vi "poc.ip.kria.generated.vi"(10 "data valid":bool[](array[boolean])=[FALSE, FALSE, TRUE, TRUE, TRUE, FALSE, FALSE, TRUE, TRUE, FALSE], 11 "ip.reset":bool[](array[boolean])=[TRUE, FALSE, FALSE, FALSE, FALSE, FALSE, FALSE, FALSE, FALSE, FALSE]) -> (1 "first word of frame":bool[](array[boolean]), 2 "recv.time (-> stream bundle)":u64[](array[numeric]), 3 "tick (counter wire -> Register write -> parser time)":u64[](array[numeric]))   [LabVIEW 2020]
doc: "REFERENCE ONLY - todo.txt item 10 (recv.time / parse.time). poc.ip.kria.vi cannot be regenerated by the AIXML tools (FIFO, Register and Timed Loop nodes are lost), so this VI shows the timestamp logic of the 156.25 MHz 'PoC IP' Timed Loop with the recommended change already made. Copy the nodes between the comment boxes into poc.ip.kria.vi; do not replace the VI.\n\nFACTS established 2026-10-11 from the AIXML export of poc.ip.kria.vi and the netlist sim of the 19:37 IP export:\n1. The tick counter (Feedback Node -> Increment -> Select, reset on the ip.reset rising edge) lives in the 156.25 MHz loop together with TDATA/TVALID/ip.reset. One tick = one 156.25 MHz cycle = 6.4 ns, NOT 10 ns (sim: recv.time advances exactly one count per input beat). Every latency figure quoted so far with 10 ns/tick is 1.56x too large.\n2. bats.parser.vi runs in the OTHER Timed Loop (100 MHz, with the CMD/DEBUG outputs). Its `time` input comes from a Register read; the Register (written with the counter every cycle in the 156 MHz loop) IS the clock-domain crossing. A wire from the counter to the parser is impossible between two Timed Loops, so the register read STAYS. Its lag (1-3 ticks, 6-19 ns) is the price of the crossing; parse.time is therefore a few ticks late, never early.\n3. Today recv.time is wired straight from the counter into the stream cluster that enters the CDC FIFO, so each CMD record carries the arrival tick of the word that completed its message (per-word stamp). The frame-start latch that existed before 2026-10-11 is gone.\n\nRECOMMENDED CHANGE (the only diagram change): put the frame-start latch back, i.e. recv.time := counter when `data valid` rises (first word of a frame), else hold the previous value. Then parse.time - recv.time is 'time since the first byte of the packet arrived', the quantity a trading system cares about, the figure is comparable with the earlier measurements, and the host tools can group a frame's records by equal recv.time. The latch is the Not / Feedback Node / And / Select / Feedback Node group in the box 'CHANGE - frame-start latch'.\n\nALTERNATIVE (no diagram change): keep the per-word stamp. Then parse.time - recv.time is the parser's own per-message latency (1 tick for a message completed by the arriving word, more for messages queued behind it) and Claude switches eval_sim.py / decode_capture.py to group by sequence number. Tell Claude which one you chose.\n\nHOST SIDE (Claude does this): TICK_NS 10 -> 6.4 in apps/poc_inject/decode_capture.py and ip_export/netlist_sim/eval_sim.py; CLAUDE.md latency figures re-stated in 6.4 ns ticks.\n\nRun this VI: ip.reset = [T,F,F,...], data valid = [F,F,T,T,T,F,F,T,T,F]. Expect tick = 0,1,2,...; first word of frame = T at indexes 2 and 7; recv.time = 0,0,2,2,2,2,2,7,7,7."
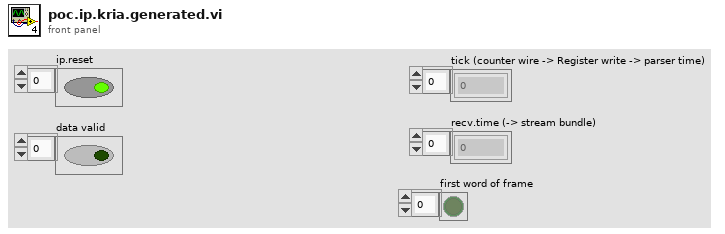
[diagram p1: front panel]
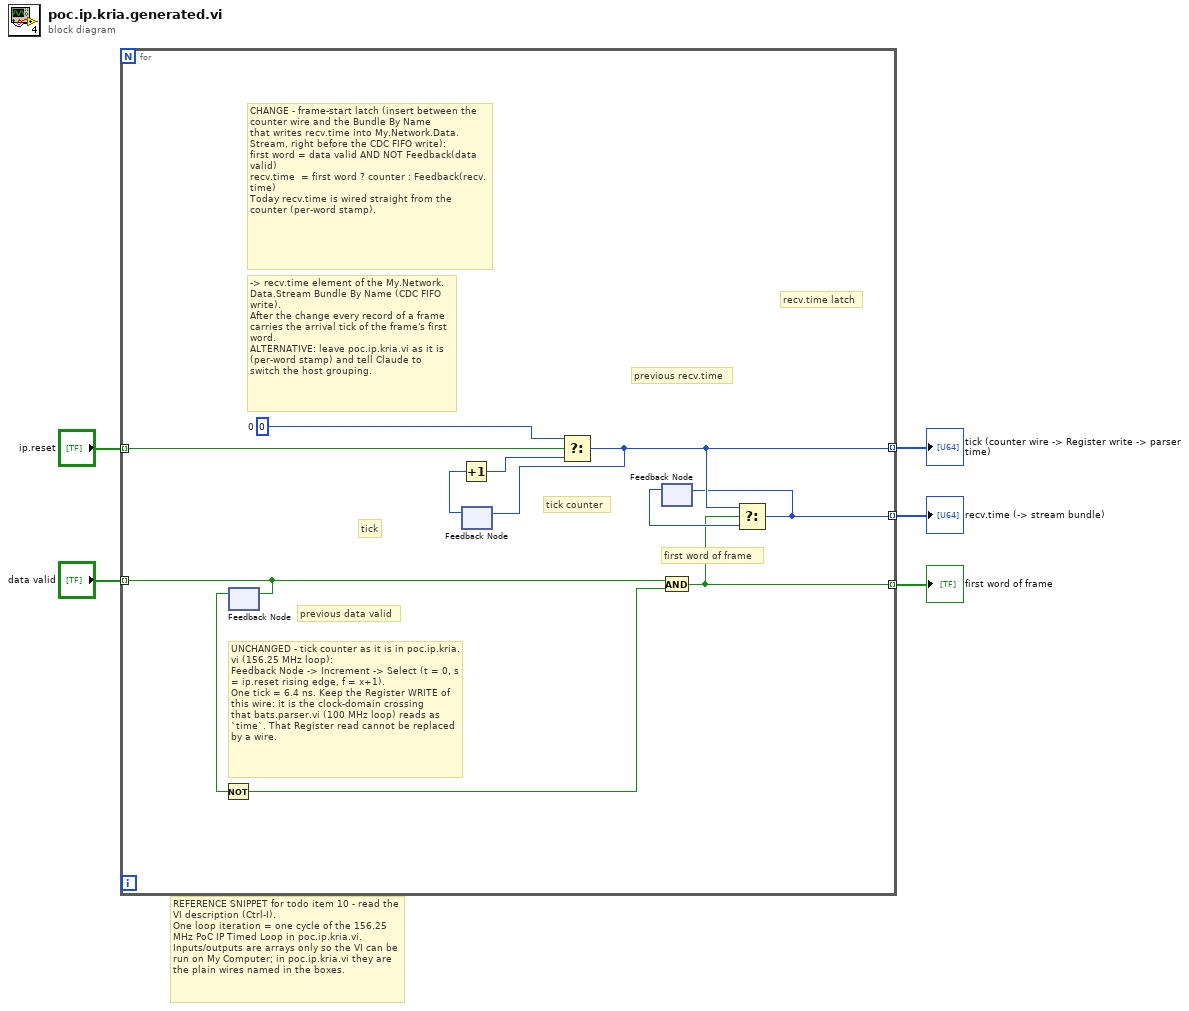
[diagram p0: block diagram]
diagram:
  # "REFERENCE SNIPPET for todo item 10 - read the VI description (Ctrl-I).\nOne loop iteration = one cycle of the 156.25 MHz PoC IP Timed Loop in poc.ip.kria.vi.\nInputs/outputs are arrays only so the VI can be run on My Computer; in poc.ip.kria.vi they are the plain wires named in the boxes."
  n1 = for {
    tunnel: "ip.reset" -> [w14] mode=indexing
    tunnel: "data valid" -> [w11] mode=indexing
    tunnel: [w8] -> w3 mode=indexing
    tunnel: [w7] -> w2 mode=indexing
    tunnel: [w6] -> w1 mode=indexing
    w15 = u64 0  # 0
    # "-> recv.time element of the My.Network.Data.Stream Bundle By Name (CDC FIFO write).\nAfter the change every record of a frame carries the arrival tick of the frame's first word.\nALTERNATIVE: leave poc.ip.kria.vi as it is (per-word stamp) and tell Claude to switch the host grouping."
    # "recv.time latch"
    # "previous recv.time"
    # "first word of frame"
    # "previous data valid"
    # "CHANGE - frame-start latch (insert between the counter wire and the Bundle By Name\nthat writes recv.time into My.Network.Data.Stream, right before the CDC FIFO write):\nfirst word = data valid AND NOT Feedback(data valid)\nrecv.time  = first word ? counter : Feedback(recv.time)\nToday recv.time is wired straight from the counter (per-word stamp)."
    # "tick counter"
    # "tick"
    # "UNCHANGED - tick counter as it is in poc.ip.kria.vi (156.25 MHz loop):\nFeedback Node -> Increment -> Select (t = 0, s = ip.reset rising edge, f = x+1).\nOne tick = 6.4 ns. Keep the Register WRITE of this wire: it is the clock-domain crossing\nthat bats.parser.vi (100 MHz loop) reads as `time`. That Register read cannot be replaced by a wire."
    n2 = feedback-in #1(w11) -> ()
    n3 = feedback #1() -> (w12:bool)  [unwired: 1 in]
    n4 = Not(x=w12) -> (.not. x?=w10:bool)
    n5 = feedback #2() -> (w16:u64)  [unwired: 1 in]
    n6 = Increment(x=w16) -> (x+1=w13:u64)
    n7 = Select(t=w15, s=w14, f=w13) -> (s? t:f=w8:u64)
    n8 = feedback-in #2(w8) -> ()
    n9 = feedback #3() -> (w9:u64)  [unwired: 1 in]
    n10 = And(x=w11, y=w10) -> (x .and. y?=w6:bool)
    n11 = Select(t=w8, s=w6, f=w9) -> (s? t:f=w7:u64)
    n12 = feedback-in #3(w7) -> ()
  }
  "tick (counter wire -> Register write -> parser time)" <- w3
  "recv.time (-> stream bundle)" <- w2
  "first word of frame" <- w1
